vi "Main Editor UI.vi"() -> ()   [LabVIEW 2015, in "SystemLink File editor node.lvclass"]
doc: "This is the main view for configuration the behavior of a module in the DCAF standard editor."
uses:
  SystemLink File editor node.lvclass
  <vilib>/NI/Configuration Framework/Node/NodeRef.ctl
  <vilib>/NI/Configuration Framework/Node/NISE_CEF_Node.lvclass
  <vilib>/NI/AMC/Message Queue.ctl
  <vilib>/NI/AMC/Message.ctl
  <vilib>/NI/Tools/Keyed Array/KeyedArray.ctl
  <vilib>/NI/Configuration Framework/Node/UserEventRef.ctl
  <vilib>/NI/Configuration Framework/Controls/EventCluster.ctl
  <vilib>/NI/Configuration Framework/Node/StopEvent.ctl
  <vilib>/NI/Configuration Framework/Node/RefreshUIEvent.ctl
  <vilib>/NI/Configuration Framework/Node/CacheState.ctl
  <vilib>/NI/Configuration Framework/Node/NodeChangeEvent.ctl
  module/configuration/Permissions Enum.ctl
  <vilib>/NI/DCAF/Tag Editor Core/Table API/Available Tag Menu/channel action event.ctl
  <vilib>/NI/DCAF/Tag Editor Core/Table API/Available Tag Menu/dialog output action.ctl
  <vilib>/NI/Tag Bus Module Framework/channel/TBM channel.lvclass
  <vilib>/NI/Tag Bus/tag/tag descriptor.lvclass
  <vilib>/NI/DCAF/Tag Editor Core/Table API/Table Manager/Call Back Ref Type Def.ctl
  <vilib>/NI/DCAF/Tag Editor Core/Configuration Editor/Classes/Engine Parent/Engine Parent Editor Node.lvclass
  <vilib>/NI/DCAF/Tag Editor Core/Configuration Editor/Classes/Module editor node/module editor node.lvclass
  module/configuration/Data Tag Type.ctl
  <vilib>/NI/DCAF/Tag Editor Core/Table API/Table Manager/references.ctl
  module/configuration/SystemLink File configuration.lvclass
  module/configuration/SystemLink File configuration.lvclass/SystemLink File configuration.ctl
  module/configuration/Read Connection Configuration.vi
  <vilib>/NI/Configuration Framework/serializable configuration/NISE_CEF_serializable configuration.lvclass
  <vilib>/NI/DCAF/Tag Editor Core/Table API/Listbox/Multi Column Listbox.lvclass
  <vilib>/NI/Configuration Framework/NISE_CEF_TreeControl.lvlib
  <vilib>/NI/Tools/Keyed Array/Tools_KeyedArray.lvlib
  <vilib>/NI/AMC/AMC.lvlib
  <vilib>/NI/DCAF/Tag Editor Core/Table API/Table Manager.lvlib
  <vilib>/NI/DCAF/Tag Editor Core/Table API/Table Manager/Table Manager.lvclass
  <vilib>/NI/DCAF UI Toolkit/Controls/DCAF UI Elements.lvlib
panel:
  in  "Top Level Tab Control":enum32{"Configuration"}(tab)
  in  "Table":i32(listbox)
  in  "Connection Type":T1(ring)
  in  "Configuration":T2={"Configuration ID"="", "HTTP"={"Verify Server?"=TRUE, "Server URL"="", "CA Certificate File"="", "User Info"={"Username"="", "Password"=""}, "API Key"=""}}
  in  "Data Type":T3
  in  "user event out":refnum<user-event>
  in  "Permissions":T4
  in  "node change":T5
  in  "cache state":T6
  in  "refresh UI":T7
  in  "stop event":T8
  in  "user event":T9
  in  "main queue":T10
  in  "node ref":T11
  # "Only AMQP is available at the moment"
  # "Enable Configuration"
  # "You can use the default value instead of a tag to always enable the transfer."
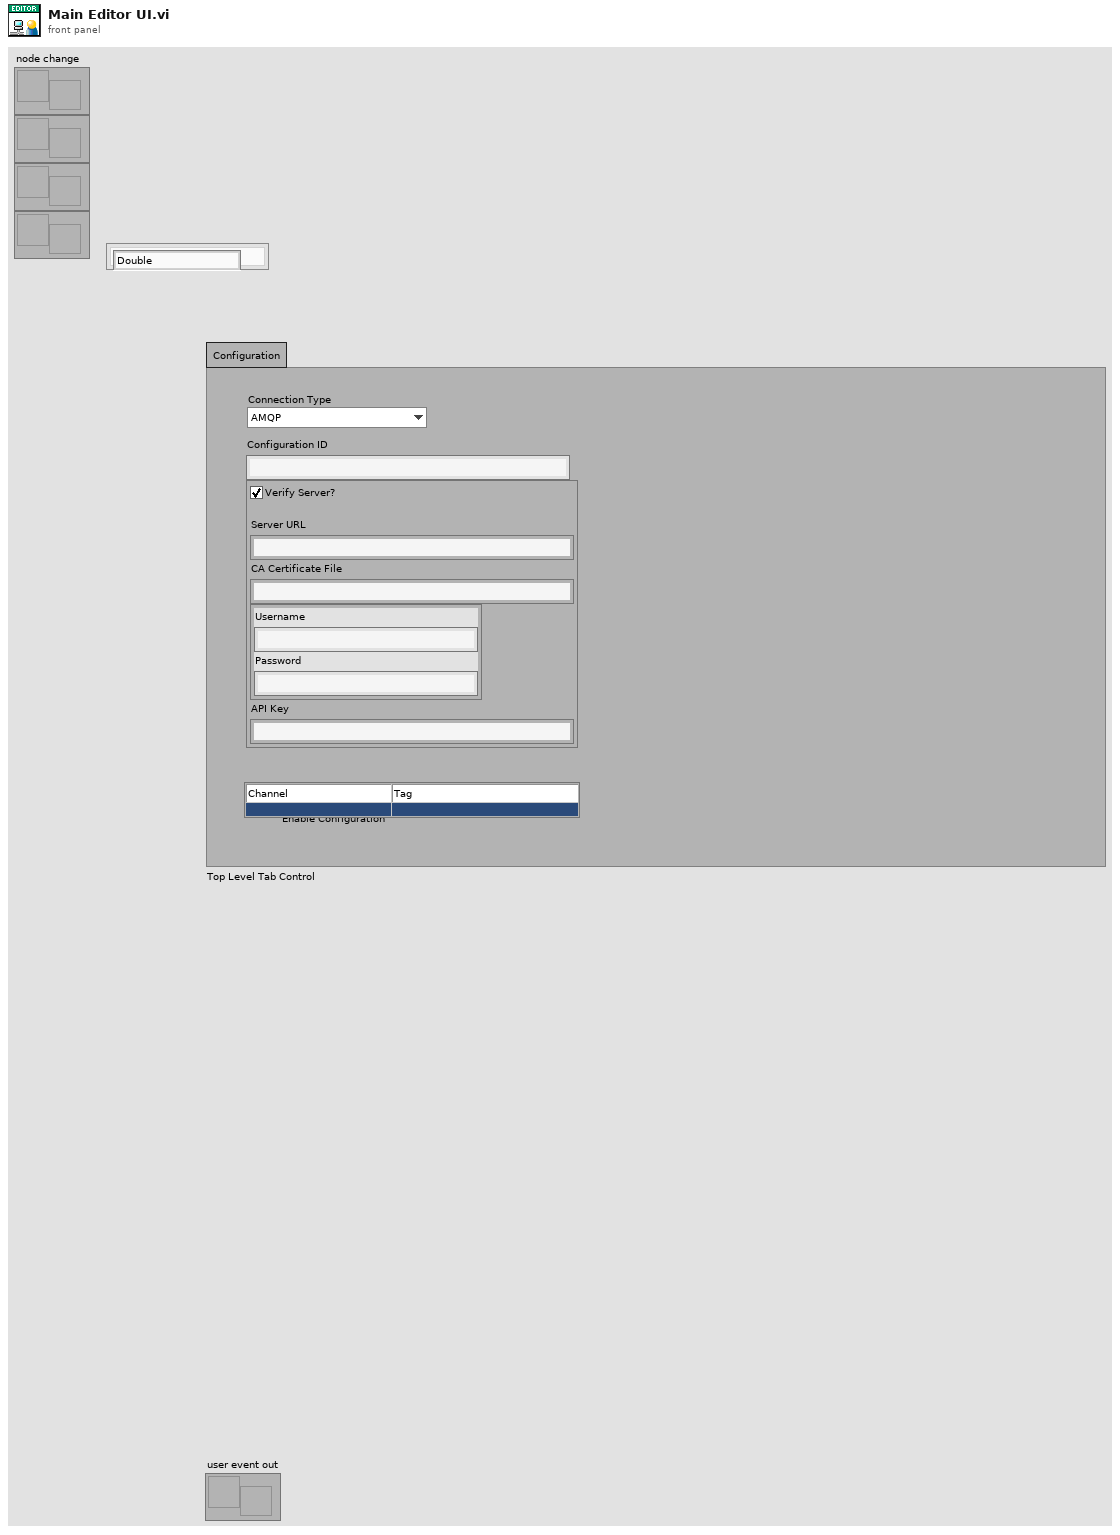
[diagram p1: front panel]
types:
  T1 = enum16{"AMQP", "HTTP", "API Key (SystemLink Cloud)"}
  T2 = cluster{"Configuration ID":string, "HTTP":cluster{"Verify Server?":bool, "Server URL":string, "CA Certificate File":string, "User Info":cluster{"Username":string, "Password":string}, "API Key":string}}
  T3 = typedef "SystemLink File configuration.lvclass/Data Tag Type.ctl" = enum16{"Double", "Single", "I32", "I16", "I8", "U64", "U32", "U16", "U8", "Boolean", "String", "Timestamp"}
  T4 = typedef "SystemLink File configuration.lvclass/Permissions Enum.ctl" = enum16{"Read from SystemLink", "Write to SystemLink"}
  T5 = typedef "NISE_CEF_Node.lvclass/NodeChangeEvent.ctl" = refnum<user-event>
  T6 = typedef "NISE_CEF_Node.lvclass/CacheState.ctl" = refnum<user-event>
  T7 = typedef "NISE_CEF_Node.lvclass/RefreshUIEvent.ctl" = refnum<user-event>
  T8 = typedef "NISE_CEF_Node.lvclass/StopEvent.ctl" = refnum<user-event>
  T9 = typedef "NISE_CEF_Node.lvclass/UserEventRef.ctl" = refnum<user-event>
  T10 = typedef "AMC.lvlib/Message Queue.ctl" = refnum<queue>
  T11 = typedef "NISE_CEF_Node.lvclass/NodeRef.ctl" = refnum<data-value>
  T12 = cluster{"AMQP Specific":refnum<vi>, "HTTP Generic":refnum<vi>, "HTTP Specific":refnum<vi>, "API Key Specific":refnum<vi>}
  T13 = typedef "Table Manager.lvlib/Table Manager.lvclass/references.ctl" = cluster{"stop event":T8, "refresh UI":T7, "cache state":T6, "node change":T5, "user event out":refnum<user-event>, "main queue":T10, "user event":T9}
  T14 = typedef "Table Manager.lvlib/Table Manager.lvclass/object ref.ctl" = cluster{"engine":refnum<data-value>, "Node Ref":refnum<data-value>}
  T15 = typedef "Table Manager.lvlib/Column.lvclass/Column Descriptor.ctl" = cluster{"name":string, "caption":string, "Column Type":T16, "Params":string, "AutoSizeMode":i32, "FillWeight":sgl, "MinWidth":u32, "tooltip":string, "Enum Reference":refnum<vi>, "Channel suffix":string, "Read Only":bool, "Call Back VI":T17, "DT Dependency":i32, "name dependency":i32, "data type":T18, "Custom Column":refnum<class "Column.lvclass">}
  T16 = typedef "Table Manager.lvlib/Column.lvclass/Column Type.ctl" = enum16{"String", "Mapping", "Enum", "Custom"}
  T17 = typedef "Table Manager.lvlib/Table Manager.lvclass/Call Back Ref Type Def.ctl" = refnum<vi>
  T18 = typedef "tag bus.lvlib/tag descriptor.lvclass/Data Type.ctl" = enum16{"Double", "Single", "I64", "I32", "I16", "I8", "U64", "U32", "U16", "U8", "Boolean", "String", "Array of Double", "Array of Single", "Array of I64", "Array of I32", "Array of I16", "Array of I8", "Array of U64", "Array of U32", "Array of U16", "Array of U8", "Array of Boolean", "Array of String"}
  T19 = typedef "SystemLink configuration.lvclass/Connection Configuration.ctl" = cluster{"Connection Type":T20, "AMQP":cluster{"Configuration ID":string}, "HTTP":cluster{"Verify Server?":bool, "Server URL":string, "CA Certificate File":string, "User Info":cluster{"Username":string, "Password":string}, "API Key":string}}
  T20 = typedef "SystemLink configuration.lvclass/Connection Type.ctl" = enum16{"AMQP", "HTTP", "API Key (SystemLink Cloud)"}
  T21 = cluster{"Verify Server?":bool, "Server URL":string, "CA Certificate File":string, "User Info":cluster{"Username":string, "Password":string}, "API Key":string}
  T22 = typedef "Table Manager.lvlib/Table Manager.lvclass/Table Events.ctl" = cluster{"Menu Selection":refnum<user-event>}
  T23 = enum8{"Enabled", "Disabled", "Disabled and Grayed Out"}
  T24 = cluster{"Configuration ID":refnum<vi>, "HTTP":refnum<vi>, "User Info":refnum<vi>, "API Key":refnum<vi>}
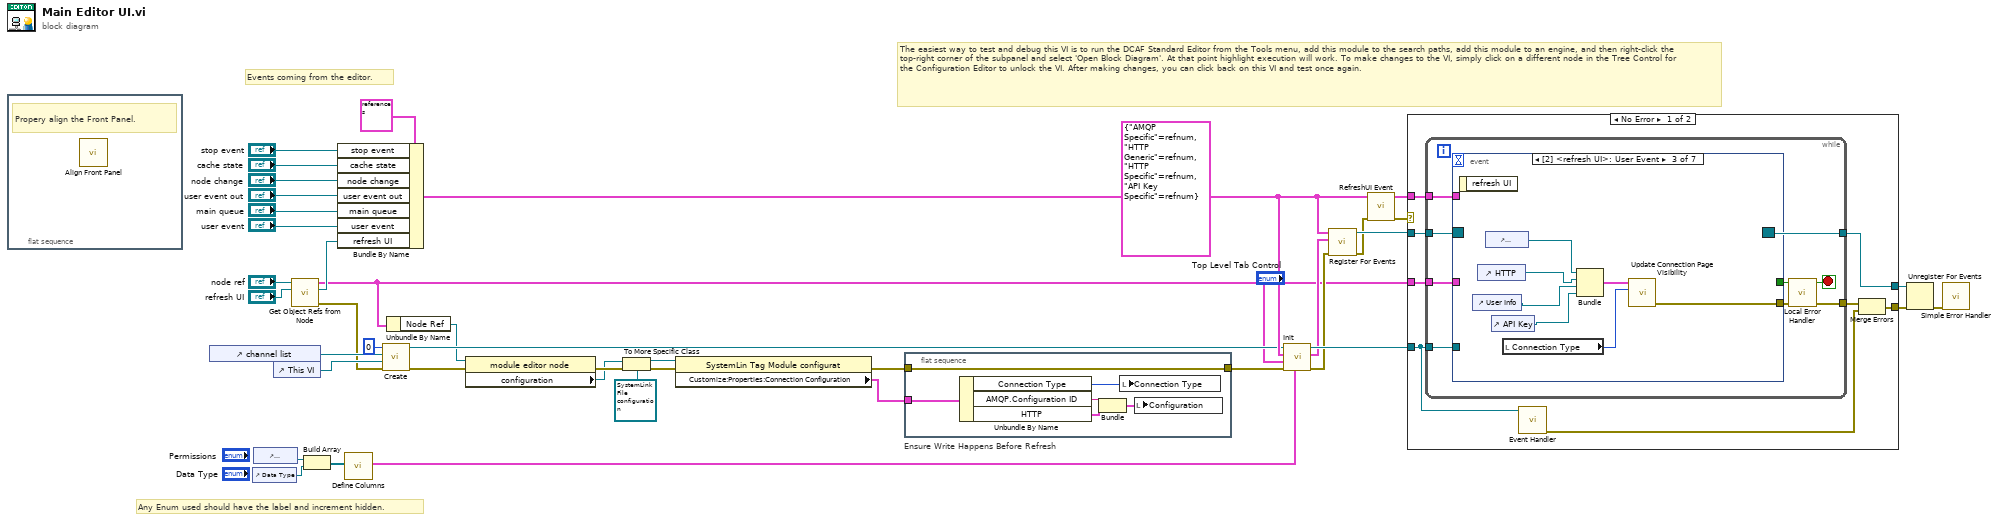
[diagram p0: block diagram]
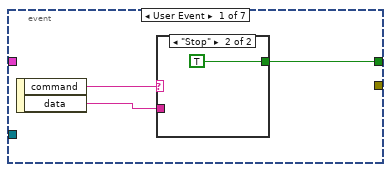
[diagram p2: hidden frame]
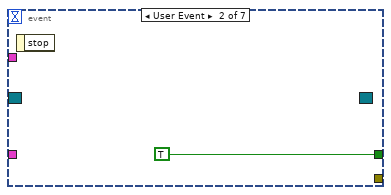
[diagram p4: hidden frame]
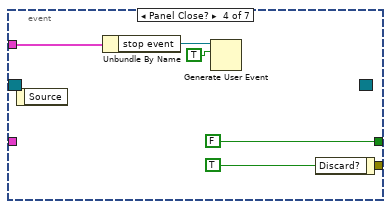
[diagram p5: hidden frame]
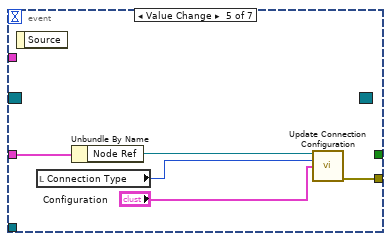
[diagram p6: hidden frame]
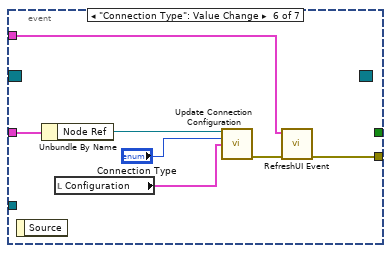
[diagram p7: hidden frame]
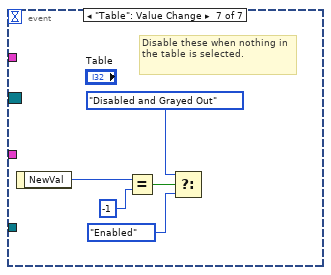
[diagram p8: hidden frame]
diagram:
  (unwired) T12 {"AMQP Specific"=refnum, "HTTP Generic"=refnum, "HTTP Specific"=refnum, "API Key Specific"=refnum} ("Config References")
  # "The easiest way to test and debug this VI is to run the DCAF Standard Editor from the Tools menu, add this module to the search paths, add this module to an engine, and then right-click the top-right corner of the subpanel and select 'Open Block Diagram'. At that point highlight execution will work. To make changes to the VI, simply click on a different node in the Tree Control for the Configuration Editor to unlock the VI. After making changes, you can click back on this VI and test once again."
  # "Any Enum used should have the label and increment hidden."
  # "Events coming from the editor."
  n1 = flat-sequence {
    frame #0 {
      # "Propery align the Front Panel."
      n2 = call <vilib>:"Align Front Panel.vi"() -> ()  [unwired: 10 in, 2 out]
    }
  }
  n3 = control-ref of="channel list"() -> (w19:refnum<vi>)
  n4 = control-ref of="Data Type"() -> (w11:refnum<vi>)
  n5 = control-ref of="Permissions"() -> (w27:refnum<vi>)
  n6 = control-ref of="This VI"() -> (w17:refnum<vi>)
  n7 = call "Get Object Refs from Node.vi"("Refresh UI"="refresh UI", "Data Value Reference in"="node ref") -> ("error out"=w14:errorcluster, "Refresh UI out"=w12:T7, "References"=w9:T14)  [unwired: 7 in]
  n8 = Build Array(w27, w11) -> (w26:refnum<vi>[])
  n9 = Bundle By Name(cluster=T13 {"stop event"=refnum, "refresh UI"=refnum, "cache state"=refnum, "node change"=refnum, "user event out"=refnum, "main queue"=refnum, "user event"=refnum} ("References"), "stop event"="stop event", "cache state"="cache state", "node change"="node change", "user event out"="user event out", "main queue"="main queue", "user event"="user event", "refresh UI"=w12) -> (w28:T13)
  n10 = call "Define Columns.vi"("Enum Array"=w26) -> ("Column Definition"=w30:T15[])  [unwired: 10 in]
  n11 = call <vilib>:"Create.vi"("error in (no error)"=w14, "Top VI"=w17, "Listbox"=w19, "Index"=0) -> ("error out"=w15:errorcluster, "reference out"=w16:refnum<class "Multi Column Listbox.lvclass">)  [unwired: 6 in]
  n12 = Unbundle By Name(w9) -> ("Node Ref"=w8:refnum<data-value>)
  n13 = property class="module editor node"(reference=w8, error in=w15) -> (error out=w10:errorcluster, "configuration"=w6:refnum<class "NISE_CEF_serializable configuration.lvclass">)  [unwired: 1 out]
  n14 = To More Specific Class(target class=refnum<class "SystemLink File configuration.lvclass"> refnum ("SystemLin Tag Module configuration"), reference=w6, error in=w10) -> (specific class reference=w4:refnum<class "SystemLink File configuration.lvclass">, error out=w7:errorcluster)
  n15 = property class="SystemLin Tag Module configurat"(reference=w4, error in=w7) -> (error out=w2:errorcluster, "Customize:Properties:Connection Configuration"=w3:T19)  [unwired: 1 out]
  n16 = flat-sequence "Ensure Write Happens Before Refresh" {
    tunnel: w3 -> [w47]
    tunnel: w2 -> [w45]
    tunnel: [w45] -> w1
    frame #0 {
      n17 = Unbundle By Name(w47) -> ("Connection Type"=w46:T20, "AMQP.Configuration ID"=w44:string, "HTTP"=w43:T21)
      n18 = Bundle("Configuration ID"=w44, "HTTP"=w43) -> (w42:T2)  [unwired: 1 in]
      n19 = local write "Connection Type"(w46) -> ()
      n20 = local write "Configuration"(w42) -> ()
    }
  }
  n21 = call-dynamic "Init.vi"("Column Descriptors"=w30, "error in (no error)"=w1, "Node object refs"=w9, "Event References"=w28, "Multi Column Listbox in"=w16) -> ("error out"=w21:errorcluster, "Table Events"=w20:T22, "Multi Column Listbox out"=w25:refnum<class "Multi Column Listbox.lvclass">)  [unwired: 4 in]
  n22 = call "Register For Events.vi"("error in"=w21, "Table Events"=w20, "References"=w28) -> ("error out"=w23:errorcluster, "Event Registration Refnum"=w31:refnum<event-registration>)  [unwired: 7 in]
  n23 = call "RefreshUI Event.vi"("error in (no error)"=w23, "References in"=w28) -> ("error out"=w22:errorcluster, "References out"=w29:T13)  [unwired: 8 in]
  n24 = case shown="No Error" w22 {
    selector: w22 -> [_ w100]
    tunnel: w31 -> [w55 w99]
    tunnel: [w54 w99] -> w41
    tunnel: [w48 w100] -> w40
    tunnel: w29 -> [w53 _]
    tunnel: w9 -> [w52 _]
    tunnel: w25 -> [w51 _]
    frame No Error {
      n25 = while {
        tunnel: w55 -> [w64]
        tunnel: [w63] -> w54
        tunnel: [w60] -> w49
        tunnel: w53 -> [w58]
        tunnel: w52 -> [w57]
        tunnel: w51 -> [w56]
        stop <- w62 stop-if-true
        n26 = event shown="[2] <refresh UI>: User Event" {
          selector: w64 -> [_ _ _ _ _ _ _]
          dyn-events: [_ _ _ _ _ _ _] -> w63
          timeout: _ -> [_ _ _ _ _ _ _]
          tunnel: [w67 TRUE _ FALSE _ _ _] -> w61
          tunnel: [_ _ w75 _ w84 w89 _] -> w59
          tunnel: w58 -> [_ _ _ w78 _ w88 _]
          tunnel: w57 -> [_ _ _ _ w86 w92 _]
          tunnel: w56 -> [_ _ _ _ _ _ _]
          event User Event {
            n27 = event-data() -> ("command"=w66:string, "data"=w65:string)  [unwired: 1 in]
            n28 = case shown="\"Stop\"" w66 {
              tunnel: [_ TRUE] -> w67
              tunnel: w65 -> [_ _]
              frame Default {
              }
              frame "Stop" {
              }
            }
          }
          event User Event {
            n29 = event-data() -> ()  [unwired: 1 in, 1 out]
          }
          event User Event {
            n30 = event-data() -> ()  [unwired: 1 in, 1 out]
            n31 = control-ref of="User Info"() -> (w73:refnum<vi>)
            n32 = control-ref of="HTTP"() -> (w70:refnum<vi>)
            n33 = control-ref of="Configuration ID"() -> (w71:refnum<vi>)
            n34 = control-ref of="API Key"() -> (w74:refnum<vi>)
            n35 = local read "Connection Type"() -> (w76:T1)
            n36 = Bundle("Configuration ID"=w71, "HTTP"=w70, "User Info"=w73, "API Key"=w74) -> (w72:T24)  [unwired: 1 in]
            n37 = call "Update Connection Page Visibility.vi"("Connection Type"=w76, "Config References"=w72) -> ("error out"=w75:errorcluster)  [unwired: 9 in]
          }
          event Panel Close? {
            n38 = event-data() -> ()  [unwired: 1 in, 1 out]
            n39 = Unbundle By Name(w78) -> ("stop event"=w77:T8)
            n40 = Generate User Event(user event=w77, event data cluster=TRUE ("event data")) -> ()  [unwired: 2 in, 2 out]
            n41 = event-data("Discard?"=TRUE) -> ()  [unwired: 1 in, 1 out]
          }
          event "Configuration.Configuration ID", "Configuration.HTTP": Value Change {
            n42 = event-data() -> ()  [unwired: 1 in, 1 out]
            n43 = local read "Connection Type"() -> (w83:T1)
            n44 = Unbundle By Name(w86) -> ("Node Ref"=w85:refnum<data-value>)
            n45 = call "Update Connection Configuration.vi"("Data Value Reference in"=w85, "Connection Type"=w83, "Configuration"="Configuration") -> ("error out"=w84:errorcluster)  [unwired: 12 in]
          }
          event "Connection Type": Value Change {
            n46 = event-data() -> ()  [unwired: 1 in, 1 out]
            n47 = Unbundle By Name(w92) -> ("Node Ref"=w93:refnum<data-value>)
            n48 = local read "Configuration"() -> (w87:T2)
            n49 = call "Update Connection Configuration.vi"("Data Value Reference in"=w93, "Connection Type"="Connection Type", "Configuration"=w87) -> ("error out"=w90:errorcluster)  [unwired: 12 in]
            n50 = call "RefreshUI Event.vi"("error in (no error)"=w90, "References in"=w88) -> ("error out"=w89:errorcluster)  [unwired: 8 in, 1 out]
          }
          event "Table": Value Change {
            # "Disable these when nothing in the table is selected."
            n51 = event-data() -> ("NewVal"=w98:i32)  [unwired: 1 in]
            n52 = Equal?(x=w98, y=-1) -> (x = y?=w96:bool)
            n53 = Select(t=T23."Disabled and Grayed Out" ("Disabled"), s=w96, f=T23."Enabled") -> ()  [unwired: 1 out]
          }
        }
        n54 = call "Local Error Handler.vi"("error in"=w59, "Stop in"=w61) -> ("error out"=w60:errorcluster, "Stop out"=w62:bool)  [unwired: 8 in]
      }
      n55 = call-dynamic "Event Handler.vi"("Listbox in"=w51) -> ("error out"=w50:errorcluster)  [unwired: 9 in, 1 out]
      n56 = Merge Errors(w49, w50) -> (w48:errorcluster)
    }
    frame Error {
    }
  }
  n57 = Unregister For Events(event registration refnum=w41, error in=w40) -> (error out=w39:errorcluster)
  n58 = call <vilib>:"Simple Error Handler.vi"("error in (no error)"=w39) -> ()  [unwired: 4 in, 5 out]
